vi "KYFG Set Grabber Value Enum By Value Name.vi"(8 "error in (no error)":errorcluster, 9 "paramValueName":string, 10 "paramName":string, 11 "handle":u32) -> (0 "error out":errorcluster, 3 "function return":u32(ring))   [LabVIEW 2023, in "KYFGLib_lv.lvlib"]
doc: "KYFG_API FGSTATUS KYFG_SetGrabberValueEnum_ByValueName(FGHANDLE handle, const char *paramName, const char *paramValueName);"
uses:
  KYFGLib_lv.lvlib
  KYFGLib.dll
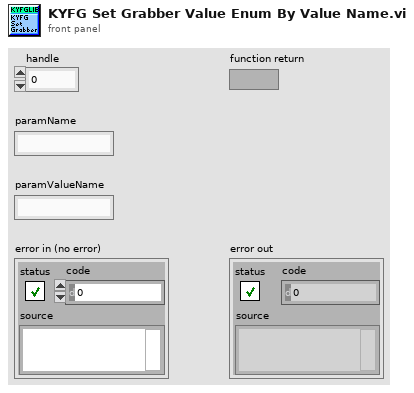
[diagram p1: front panel]
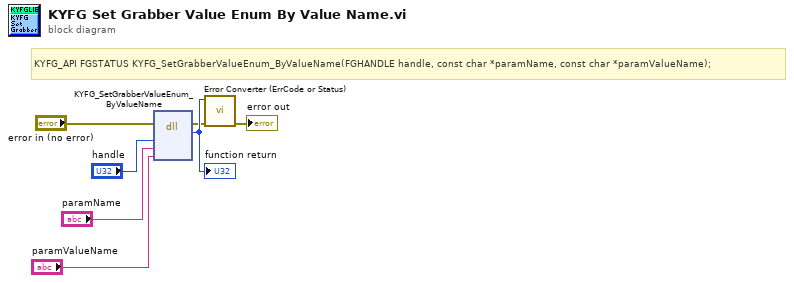
[diagram p0: block diagram]
diagram:
  # "KYFG_API FGSTATUS\tKYFG_SetGrabberValueEnum_ByValueName(FGHANDLE handle, const char *paramName, const char *paramValueName);"
  n1 = dll-call lib="KYFGLib.dll" fn="KYFG_SetGrabberValueEnum_ByValueName"(error in="error in (no error)", "handle"="handle", "paramName"="paramName", "paramValueName"="paramValueName") -> (error out=w2:errorcluster, "return type"=w7:u32)  [unwired: 5 in, 1 out]
  "function return" <- w7
  n2 = call "Error Converter (ErrCode or Status).vi"("error in (no error)"=w2, "error code"=w7) -> ("error out"=→"error out":errorcluster)  [unwired: 9 in]
